vi "query Measurement Window Mode - FSV40.vi"(8 "error in (no error)":errorcluster, 10 "Measurement Window Mode":T1, 11 "FSV-40N in":refnum<class "FSV-40N.lvclass">) -> (0 "error out":errorcluster, 2 "Measurement Value Array":dbl[](array[numeric]), 3 "FSV-40N out":refnum<class "FSV-40N.lvclass">)   [LabVIEW 2023, in "Spectrum Analyzer.lvlib" / "FSV-40N.lvclass"]
uses:
  FSV-40N.lvclass
  FSV-40N.lvclass/FSV-40N.ctl
  Spectrum Analyzer.lvlib
  TYPE DEFINITION/TYPE Measurement Window Mode.ctl
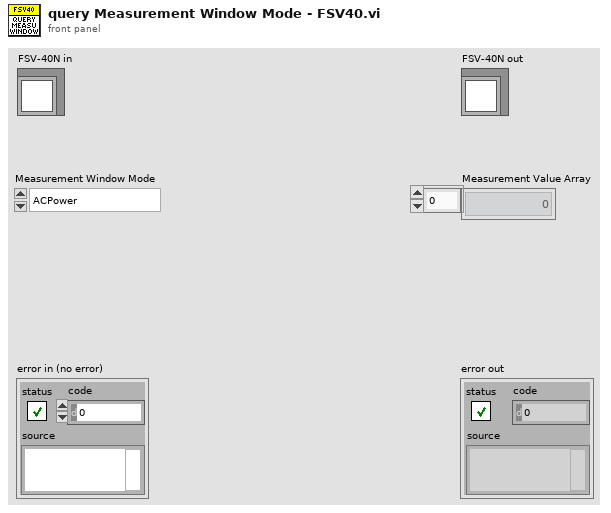
[diagram p1: front panel]
types:
  T1 = typedef "Spectrum Analyzer.lvlib/TYPE Measurement Window Mode.ctl" = enum16{"ACPower", "CPOWer", "MCACpower", "OBANdwidth", "OBWidth", "CN", "CN0"}
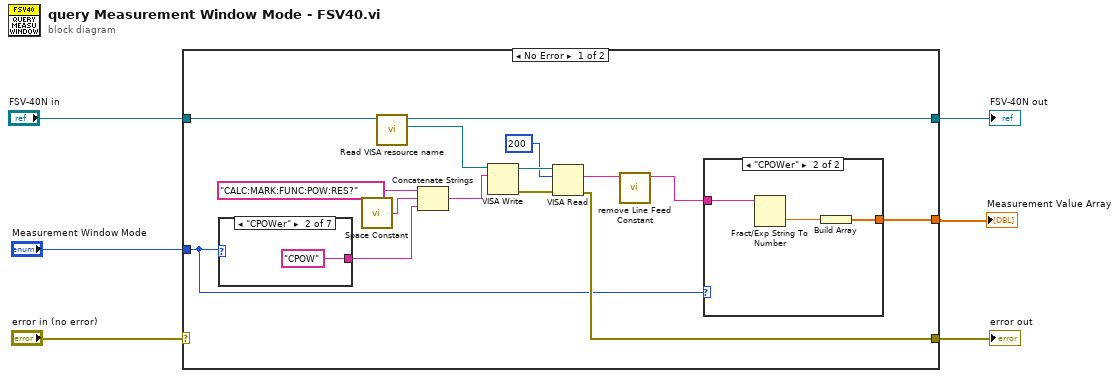
[diagram p0: block diagram]
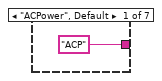
[diagram p3: hidden frame]
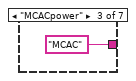
[diagram p4: hidden frame]
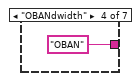
[diagram p5: hidden frame]
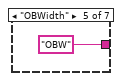
[diagram p6: hidden frame]
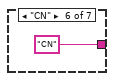
[diagram p7: hidden frame]
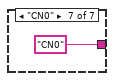
[diagram p8: hidden frame]
diagram:
  n1 = case shown="No Error" "error in (no error)" {
    selector: "error in (no error)" -> [_ w32]
    tunnel: "FSV-40N in" -> [w21 w33]
    tunnel: [w15 w33] -> w5
    tunnel: [w11 w32] -> w3
    tunnel: "Measurement Window Mode" -> [w8 _]
    tunnel: [w7 _] -> w1
    frame No Error {
      n2 = case shown="\"CPOWer\"" w8 {
        tunnel: ["ACP" "CPOW" "MCAC" "OBAN" "OBW" "CN" "CN0"] -> w18
        frame "ACPower", Default {
        }
        frame "CPOWer" {
        }
        frame "MCACpower" {
        }
        frame "OBANdwidth" {
        }
        frame "OBWidth" {
        }
        frame "CN" {
        }
        frame "CN0" {
        }
      }
      n3 = call <vilib>:"Space Constant.vi"() -> ("String"=w19:string)
      n4 = call "Read VISA resource name.vi"("FSV-40N in"=w21) -> ("VISA resource name"=w17:refnum<visa-resource-name>, "FSV-40N out"=w15:refnum<class "FSV-40N.lvclass">)  [unwired: 8 in, 1 out]
      n5 = Concatenate Strings("CALC:MARK:FUNC:POW:RES?" ("string"), w19, w18) -> (w16:string)
      n6 = VISA Write(VISA resource name=w17, write buffer=w16) -> (VISA resource name out=w14:refnum<visa-resource-name>, error out=w13:errorcluster)  [unwired: 1 in, 1 out]
      n7 = VISA Read(VISA resource name=w14, byte count=u32 200, error in (no error)=w13) -> (read buffer=w10:string, error out=w11:errorcluster)  [unwired: 2 out]
      n8 = call "remove Line Feed Constant.vi"("Input String"=w10) -> ("Line Feed Removed String"=w9:string)  [unwired: 10 in]
      n9 = case shown="\"CPOWer\"" w8 {
        tunnel: w9 -> [_ w24]
        tunnel: [_ w22] -> w7
        frame "ACPower", Default {
        }
        frame "CPOWer" {
          n10 = Fract/Exp String To Number(string=w24) -> (number=w23:dbl)  [unwired: 3 in, 1 out]
          n11 = Build Array(w23) -> (w22:dbl[])
        }
      }
    }
    frame Error {
    }
  }
  "error out" <- w3
  "FSV-40N out" <- w5
  "Measurement Value Array" <- w1
